vi "Tick.vi"(8 "error in":errorcluster, 11 "VTU Sim Rig in":refnum<class "VTU Sim Rig.lvclass">) -> (0 "error out":errorcluster, 3 "VTU Sim Rig out":refnum<class "VTU Sim Rig.lvclass">)   [LabVIEW 2026, in "VTU Sim Rig.lvclass"]
doc: "One 100 ms tick of the simulated rig: integrates State toward Setpoints with Sim First Order Step (dt 0.1), stores the new State, builds the Channel Feedback value (channels = new State, timestamp_ms = Tick Count ms) and publishes it through Publish Feedback. Message: Tick Msg."
uses:
  VTU Sim Rig.lvclass
  VTU Sim Rig.lvclass/VTU Sim Rig.ctl
  src/Rig/Rig.lvclass
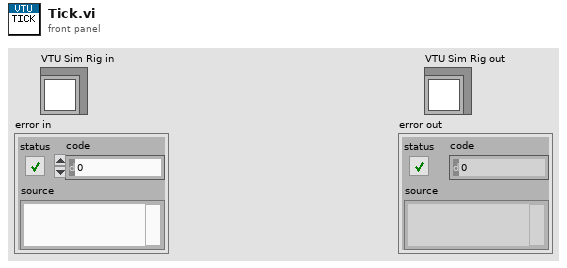
[diagram p1: front panel]
types:
  T1 = cluster{"channels":cluster{"channel":string, "value":dbl}[], "timestamp_ms":dbl}
  T2 = typedef "Channel Value.ctl" = cluster{"channel":string, "value":dbl}
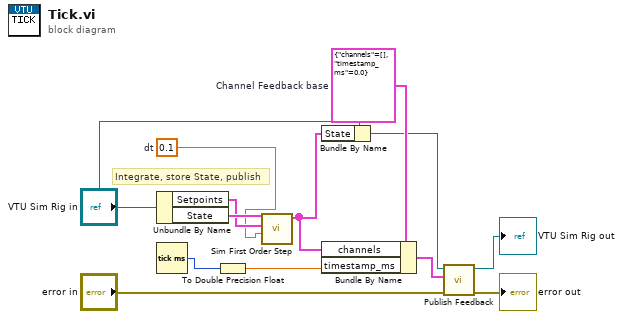
[diagram p0: block diagram]
diagram:
  w6 = T1 {"channels"=[], "timestamp_ms"=0.0}  # Channel Feedback base
  w11 = 0.1  # dt
  # "Integrate, store State, publish"
  n1 = Unbundle By Name("VTU Sim Rig in") -> ("Setpoints"=w12:T2[], "State"=w13:T2[])
  n2 = Tick Count (ms)() -> (millisecond timer value=w9:u32)
  n3 = To Double Precision Float(number=w9) -> (double precision float=w7:dbl)
  n4 = call "Sim First Order Step.vi"("dt s"=w11, "Setpoints"=w12, "State"=w13) -> ("new State"=w8:T2[])  [unwired: 8 in]
  n5 = Bundle By Name(cluster="VTU Sim Rig in", "State"=w8) -> (w5:refnum<class "VTU Sim Rig.lvclass">)
  n6 = Bundle By Name(cluster=w6, "channels"=w8, "timestamp_ms"=w7) -> (w4:T1)
  n7 = call "Publish Feedback.vi"("error in"="error in", "Channel Feedback"=w4, "Rig in"=w5) -> ("error out"=→"error out":errorcluster, "Rig out"=→"VTU Sim Rig out":refnum<class "VTU Sim Rig.lvclass">)  [unwired: 7 in]
